vi "Command and read pump.vi"(8 "error in (no error)":errorcluster, 9 "command":string, 10 "Address (00)":i32, 11 "VISA resource name":refnum<visa-resource-name>) -> (0 "error out":errorcluster, 1 "Output String":string, 2 "Pump status":T2 items=["Error - Can't read status"=-1, "Stopped"=0, "Infusing"=1, "Withdrawing"=2, "Pump stalled"=3, "Stopped at infuse limit"=4, "Stopped at withdraw limit"=5, "Emergency stop"=6, "Stopped at target volume"=7], 3 "VISA resource name out":refnum<visa-resource-name>, 4 "Numeric result":dbl, 5 "String result":string)   [LabVIEW 2015]
doc: "This VI sends a specificed commnd to the pump and returns the pump response and status.\n\nModified from original which is Copyright 2005, National Instruments Corporation.\n\nModifications Copyright 2009, Jeff Gelles, Brandeis University"
uses:
  Pump status.ctl
panel:
  in  "Log":enum16{"None", "All", "Error only"}(ring)
  in  "Log":T1(array[cluster])
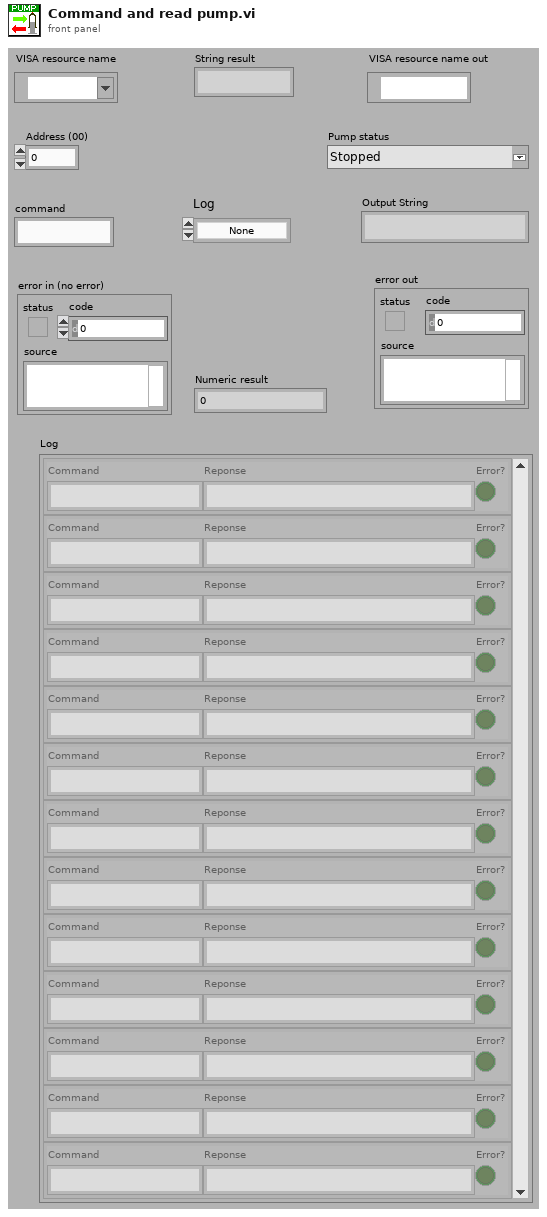
[diagram p1: front panel]
types:
  T1 = cluster{"Command":string, "Reponse":string, "Error?":bool}[]
  T2 = typedef "Pump status.ctl" = i8
  T3 = cluster{"command":string, "Output String":string, "status":bool}
  T4 = cluster{"command":string, "Output String":string, "status":bool}[]
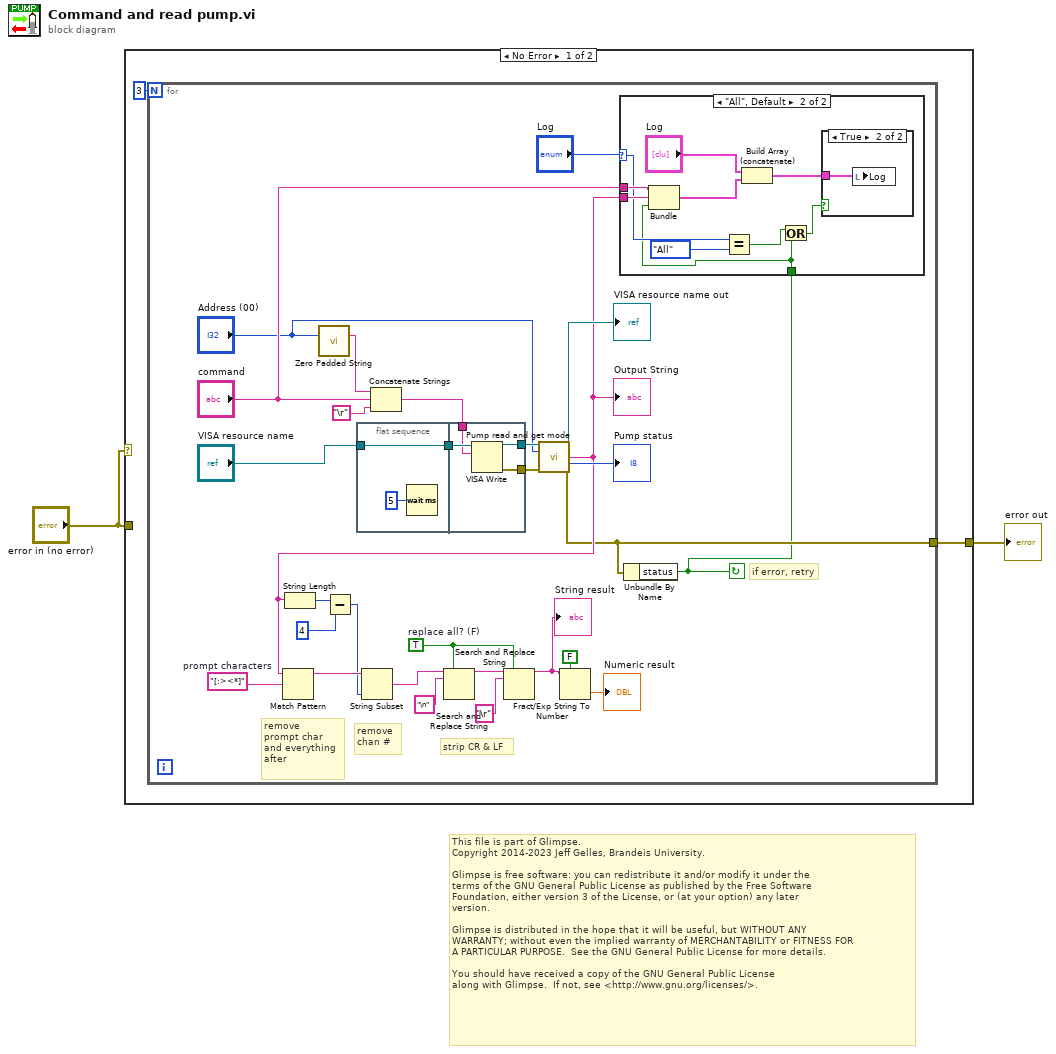
[diagram p0: block diagram]
diagram:
  # "This file is part of Glimpse. \nCopyright 2014-2023 Jeff Gelles, Brandeis University.    \n\nGlimpse is free software: you can redistribute it and/or modify it under the \nterms of the GNU General Public License as published by the Free Software \nFoundation, either version 3 of the License, or (at your option) any later \nversion.\n\nGlimpse is distributed in the hope that it will be useful, but WITHOUT ANY \nWARRANTY; without even the implied warranty of MERCHANTABILITY or FITNESS FOR \nA PARTICULAR PURPOSE.  See the GNU General Public License for more details.\n\nYou should have received a copy of the GNU General Public License\nalong with Glimpse.  If not, see <http://www.gnu.org/licenses/>."
  n1 = case shown="No Error" "error in (no error)" {
    tunnel: [w4 w50] -> w2
    tunnel: "error in (no error)" -> [_ w50]
    frame No Error {
      n2 = for {
        N: 3 -> [_]
        tunnel: [w8] -> w4
        stop <- w6 continue-if-true
        w5 = TRUE  # replace all? (F)
        w23 = "[:><*]"  # prompt characters
        # "if error, retry"
        # "strip CR & LF"
        # "remove \nchan #"
        # "remove \nprompt char\nand everything\nafter"
        n3 = call "Zero Padded String.vi"("Address (00)"="Address (00)") -> ("Zero Padded Address String"=w24:string)  [unwired: 14 out]
        n4 = flat-sequence {
          tunnel: "VISA resource name" -> [w45]
          tunnel: [w45] -> w32
          tunnel: [w49] -> w28
          tunnel: [w48] -> w27
          tunnel: w25 -> [w46]
          tunnel: w32 -> [w47]
          frame #0 {
            n5 = Wait (ms)(milliseconds to wait=u32 5) -> ()  [unwired: 1 out]
          }
          frame #1 {
            n6 = VISA Write(VISA resource name=w47, write buffer=w46) -> (VISA resource name out=w49:refnum<visa-resource-name>, error out=w48:errorcluster)  [unwired: 1 in, 1 out]
          }
        }
        n7 = Concatenate Strings(w24, "command", "\r") -> (w25:string)
        n8 = call "Pump read and get mode.vi"("VISA resource name"=w28, "Address (00)"="Address (00)", "error in (no error)"=w27) -> ("VISA resource name out"=→"VISA resource name out":refnum<visa-resource-name>, "Output String"=w10:string, "Pump status"=→"Pump status":T2, "error out"=w8:errorcluster)  [unwired: 9 out]
        "Output String" <- w10
        n9 = Match Pattern(string=w10, regular expression=w23) -> (before substring=w22:string)  [unwired: 4 out]
        n10 = String Length(string=w10) -> (length=w21:i32)
        n11 = Subtract(x=w21, y=4) -> (x-y=w19:i32)
        n12 = String Subset(string=w22, length (rest)=w19) -> (substring=w18:string)  [unwired: 1 out]
        n13 = Search and Replace String(replace all?=w5, input string=w18, search string="\n") -> (result string=w15:string)  [unwired: 1 in, 7 out]
        n14 = Search and Replace String(replace all?=w5, input string=w15, search string="\r") -> (result string=w12:string)  [unwired: 1 in, 7 out]
        "String result" <- w12
        n15 = Fract/Exp String To Number(use system decimal point (T)=FALSE, string=w12) -> (number=→"Numeric result":dbl)  [unwired: 3 out]
        n16 = Unbundle By Name(w8) -> ("status"=w6:bool)
        n17 = case shown="\"All\", Default" "Log" {
          selector: "Log" -> [_ w35]
          tunnel: "command" -> [_ w42]
          tunnel: w10 -> [_ w41]
          tunnel: w6 -> [_ w33]
          frame "None" {
          }
          frame "All", Default {
            n18 = Bundle("command"=w42, "Output String"=w41, "status"=w33) -> (w39:T3)  [unwired: 1 out]
            n19 = Equal?(x=w35, y=enum16{"None", "All", "Error only"}."All") -> (x = y?=w36:bool)
            n20 = Build Array (concatenate)("Log", w39) -> (w38:T4)
            n21 = Or(x=w36, y=w33) -> (x .or. y?=w37:bool)
            n22 = case shown="True" w37 {
              tunnel: w38 -> [_ w43]
              frame False {
              }
              frame True {
                n23 = local write "Log"(w43) -> ()
              }
            }
          }
        }
      }
    }
    frame Error {
    }
  }
  "error out" <- w2
